vi "Parse List Objects Result.vi"(8 "error in (no error)":errorcluster, 10 "Response body":string) -> (0 "error out":errorcluster, 3 "List Objects Result":T1)   [LabVIEW 2015, in "NI_AWS_S3.lvlib" / "Object.lvlib"]
doc: "Parse out the Results from the Response body of a List bucket request."
uses:
  Object.lvlib
  List Objects Result.ctl
  Object Content.ctl
  Storage Class.ctl
  Owner.ctl
  NI_AWS_S3.lvlib
  XML Parsing/NI_XML Parsing.lvlib
  Core/NI_AWS_Core.lvlib
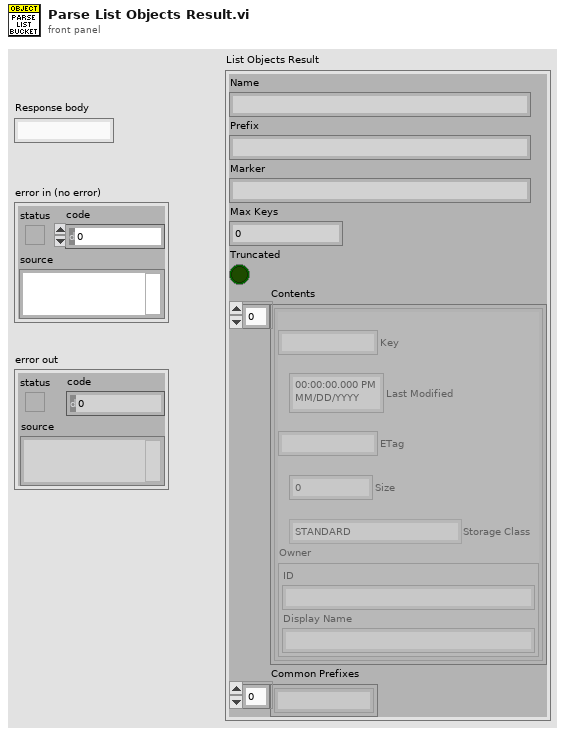
[diagram p1: front panel]
types:
  T1 = typedef "NI_AWS_S3.lvlib/List Objects Result.ctl" = cluster{"Name":string, "Prefix":string, "Marker":string, "Max Keys":u16, "Truncated":bool, "Contents":T2[], "Common Prefixes":string[]}
  T2 = typedef "NI_AWS_S3.lvlib/Object Content.ctl" = cluster{"Key":string, "Last Modified":timestamp, "ETag":string, "Size":u64, "Storage Class":T3, "Owner":T4}
  T3 = typedef "NI_AWS_S3.lvlib/Storage Class.ctl" = enum16{"STANDARD", "REDUCED_REDUNDANCY"}
  T4 = typedef "NI_AWS_S3.lvlib/Owner.ctl" = cluster{"ID":string, "Display Name":string}
  T5 = cluster{"[0]":string, "[1]":string, "[2]":string, "[3]":string, "[4]":string}
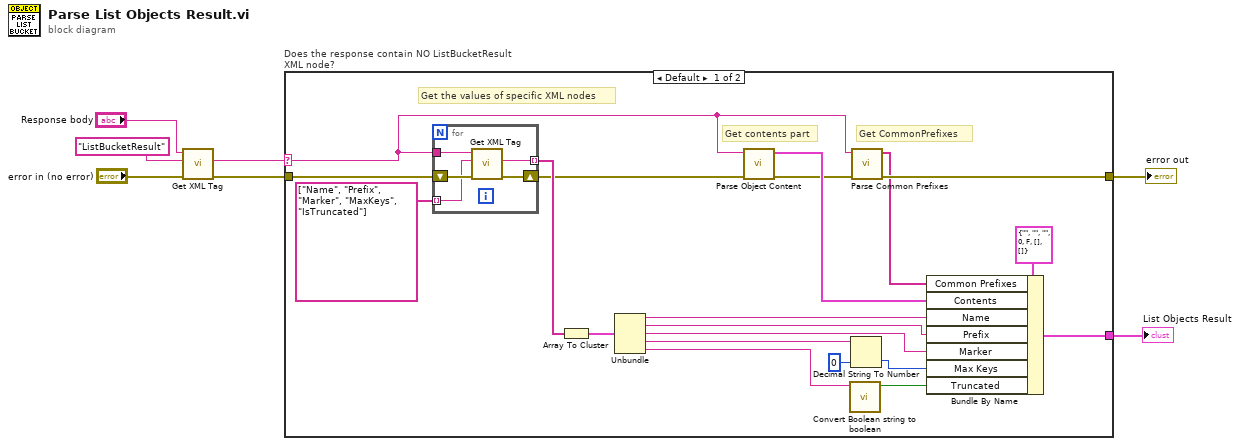
[diagram p0: block diagram]
diagram:
  n1 = call "Get XML Tag.vi"("error in (no error)"="error in (no error)", "Tag name"="ListBucketResult", "XML String in"="Response body") -> ("error out"=w2:errorcluster, "Tag value"=w1:string)  [unwired: 4 in, 3 out]
  n2 = case "Does the response contain NO ListBucketResult XML node?" shown="Default" w1 {
    selector: w1 -> [w8 _]
    tunnel: w2 -> [w19 w33]
    tunnel: [w26 _] -> w7
    tunnel: [w23 w33] -> w6
    frame Default {
      # "Get the values of specific XML nodes"
      # "Get CommonPrefixes"
      # "Get contents part"
      n3 = for {
        tunnel: string[] ["Name", "Prefix", "Marker", "MaxKeys", "IsTruncated"] -> [w31] mode=indexing
        tunnel: w8 -> [w30]
        tunnel: [w29] -> w18 mode=indexing
        shift-right: [w28] -> w9
        shift-left: w19 -> [w32]
        n4 = call "Get XML Tag.vi"("error in (no error)"=w32, "Tag name"=w31, "XML String in"=w30) -> ("error out"=w28:errorcluster, "Tag value"=w29:string)  [unwired: 4 in, 3 out]
      }
      n5 = Array To Cluster(array=w18) -> (cluster=w17:T5)
      n6 = Unbundle(w17) -> ("[0]"=w16:string, "[1]"=w15:string, "[2]"=w14:string, "[3]"=w13:string, "[4]"=w11:string)
      n7 = call "Parse Object Content.vi"("error in (no error)"=w9, "Response body"=w8) -> ("error out"=w24:errorcluster, "Object content"=w25:T2[])  [unwired: 8 in]
      n8 = call "Convert Boolean string to boolean.vi"("Boolean String"=w11) -> ("Boolean"=w10:bool)  [unwired: 10 in]
      n9 = Decimal String To Number(string=w13, default (0L)=u16 0) -> (number=w12:u16)  [unwired: 1 in, 1 out]
      n10 = call "Parse Common Prefixes.vi"("error in (no error)"=w24, "Response body"=w8) -> ("error out"=w23:errorcluster, "Common Prefixes"=w22:string[])  [unwired: 8 in]
      n11 = Bundle By Name(cluster=T1 {"Name"="", "Prefix"="", "Marker"="", "Max Keys"=0, "Truncated"=FALSE, "Contents"=[], "Common Prefixes"=[]} ("List Objects Result"), "Common Prefixes"=w22, "Contents"=w25, "Name"=w16, "Prefix"=w15, "Marker"=w14, "Max Keys"=w12, "Truncated"=w10) -> (w26:T1)
    }
    frame "" {
      # "Something bad happened, as the necessary info is not here, so do nothing!"
    }
  }
  "List Objects Result" <- w7
  "error out" <- w6
